vi "Reconfig ECAT Modules.vi"(8 "error in (no error)":errorcluster) -> (0 "error out":errorcluster)   [LabVIEW 2027, in "SEECD Engine.lvlib"]
uses:
  SEECD Engine.lvlib
  Type Defs/ECAT Reconfig State.ctl
  Includes/Modules.lvlibp/RSI Module/RSI Module.lvclass
  <vilib>/NI VeriStand/Custom Device Tools/Custom Device Utility Library/Custom Device Utility Library.lvlib
  Type Defs/ECAT Module Reconfig.ctl
  Type Defs/ECAT Reconfig Status.ctl
panel:
  in  "Status":refnum<queue>
  in  "ECAT Modules":T1[](array[typedef])
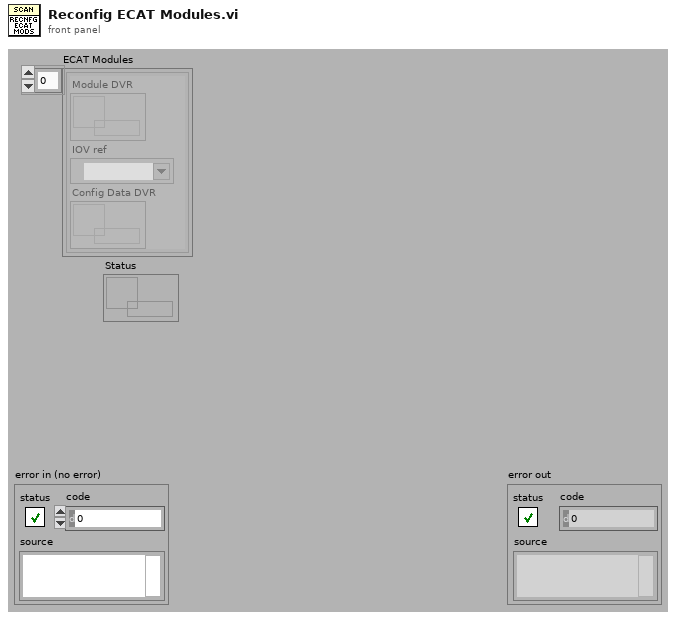
[diagram p1: front panel]
types:
  T1 = typedef "SEECD Engine.lvlib/ECAT Module Reconfig.ctl" = cluster{"Module DVR":refnum<data-value>, "IOV ref":refnum<k21>, "Config Data DVR":refnum<data-value>}
  T2 = typedef "SEECD Engine.lvlib/ECAT Reconfig State.ctl" = enum16{"Not running", "Waiting to Start", "Started", "Running"}
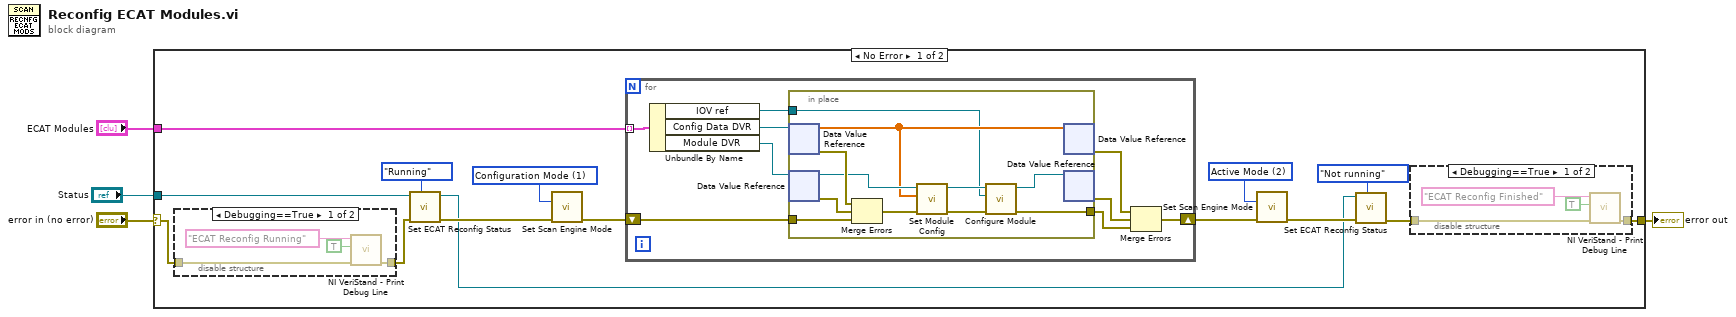
[diagram p0: block diagram]
diagram:
  n1 = case shown="No Error" "error in (no error)" {
    selector: "error in (no error)" -> [w6 w50]
    tunnel: "ECAT Modules" -> [w19 _]
    tunnel: [w7 w50] -> w2
    tunnel: "Status" -> [w13 _]
    frame No Error {
      w15 = 2 items=["Configuration Mode"=1, "Active Mode"=2] ("mode (Active Mode)")
      w18 = 1 items=["Configuration Mode"=1, "Active Mode"=2] ("mode (Active Mode)")
      n2 = disable-structure shown="Debugging==True" {
        disable-tunnel: w6 -> [w27 w29]
        disable-tunnel: [w26 w29] -> w5
        frame condition #0 {
          n3 = call <vilib>:"NI VeriStand - Print Debug Line.vi"("error in (no error)"=w27, "Add to log file? (F)"=TRUE, "Message"="ECAT Reconfig Running" ("String to write")) -> ("error out"=w26:errorcluster)  [unwired: 8 in]
        }
        frame condition #1 (active) {
        }
      }
      n4 = call "Set ECAT Reconfig Status.vi"("State"=ECAT_Reconfig_State."Running", "error in (no error)"=w5, "Status in"=w13) -> ("error out"=w14:errorcluster, "Status out"=w9:refnum<queue>)  [unwired: 7 in]
      n5 = call <vilib>:"Set Scan Engine Mode.vi"("mode (Active Mode)"=w18, "error in (no error)"=w14) -> ("error out"=w17:errorcluster)  [unwired: 13 in]
      n6 = for {
        tunnel: w19 -> [w38] mode=indexing
        shift-right: [w33] -> w16
        shift-left: w17 -> [w35]
        n7 = Unbundle By Name(w38) -> ("IOV ref"=w34:refnum<k21>, "Config Data DVR"=w37:refnum<data-value>, "Module DVR"=w36:refnum<data-value>)
        n8 = in-place {
          in-place-border: w35 -> [w49]
          in-place-border: w34 -> [w39]
          in-place-border: [w40] -> w30
          n9 = in-place-dvr #1(w37) -> (w41:dbl[], w47:errorcluster)
          n10 = in-place-dvr #2(w36) -> (w43:refnum<class "RSI Module.lvclass">, w48:errorcluster)
          n11 = Merge Errors(w47, w48, w49) -> (w44:errorcluster)
          n12 = call-dynamic "Set Module Config.vi"("error in (no error)"=w44, "Config Channels"=w41, "RSI Module in"=w43) -> ("error out"=w45:errorcluster, "RSI Module out"=w46:refnum<class "RSI Module.lvclass">)  [unwired: 7 in]
          n13 = call-dynamic "Configure Module.vi"("error in (no error)"=w45, "IOV ref in"=w39, "RSI Module in"=w46) -> ("error out"=w40:errorcluster, "RSI Module out"=w42:refnum<class "RSI Module.lvclass">)  [unwired: 6 in, 1 out]
          n14 = in-place-dvr #1(w41) -> (w32:errorcluster)  [unwired: 1 out]
          n15 = in-place-dvr #2(w42) -> (w31:errorcluster)  [unwired: 1 out]
        }
        n16 = Merge Errors(w32, w31, w30) -> (w33:errorcluster)
      }
      n17 = call <vilib>:"Set Scan Engine Mode.vi"("mode (Active Mode)"=w15, "error in (no error)"=w16) -> ("error out"=w10:errorcluster)  [unwired: 13 in]
      n18 = call "Set ECAT Reconfig Status.vi"("State"=ECAT_Reconfig_State."Not running", "error in (no error)"=w10, "Status in"=w9) -> ("error out"=w8:errorcluster)  [unwired: 7 in, 1 out]
      n19 = disable-structure shown="Debugging==True" {
        disable-tunnel: w8 -> [w22 w24]
        disable-tunnel: [w21 w24] -> w7
        frame condition #0 {
          n20 = call <vilib>:"NI VeriStand - Print Debug Line.vi"("error in (no error)"=w22, "Add to log file? (F)"=TRUE, "Message"="ECAT Reconfig Finished" ("String to write")) -> ("error out"=w21:errorcluster)  [unwired: 8 in]
        }
        frame condition #1 (active) {
        }
      }
    }
    frame Error {
    }
  }
  "error out" <- w2
